vi "Close.vi"(8 "error in (no error)":errorcluster, 11 "DBC in":refnum<class "DBC.lvclass">) -> (0 "error out":errorcluster)   [LabVIEW 2020, in "ORM_pgsql_jdp.lvlib" / "DBC.lvclass"]
uses:
  DBC.lvclass
  DBC.lvclass/DBC.ctl
  <vilib>/Viviota/shared/ORM.lvlibp/DbConnection/DbConnection.lvclass
  <vilib>/JDP Science/PostgreSQL Library/Connection/PQ Connection.lvclass
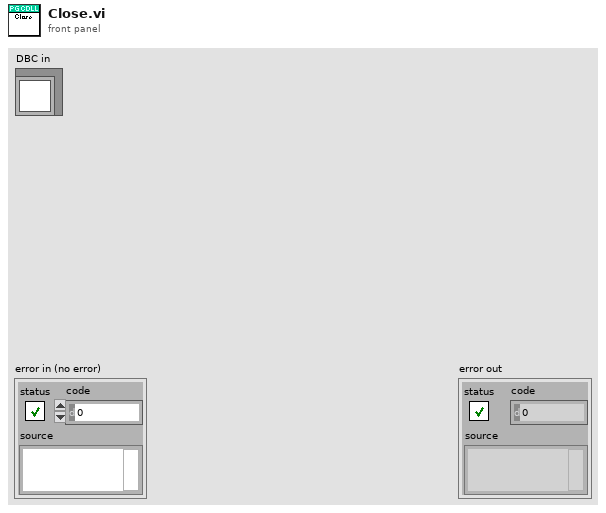
[diagram p1: front panel]
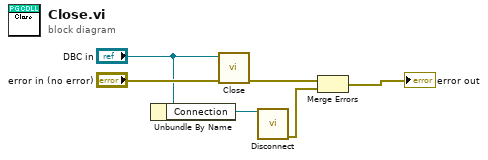
[diagram p0: block diagram]
diagram:
  n1 = Unbundle By Name("DBC in") -> ("Connection"=w3:refnum<class "PQ Connection.lvclass">)
  n2 = call-parent "Close.vi"("error in (no error)"="error in (no error)", "DbConnection in"="DBC in") -> ("error out"=w6:errorcluster)  [unwired: 9 in]
  n3 = call <vilib>:"Disconnect.vi"("PQ Connection in"=w3) -> ("error out"=w1:errorcluster)  [unwired: 10 in]
  n4 = Merge Errors(w6, w1) -> (→"error out":errorcluster)
